vi "Place New Object After ID Object.vi"(7 "Named Cluster":variant, 8 "Identifying Attribute Value":string, 9 "Identifying Attribute Type":string, 10 "Element Type":string, 11 "XML String":string) -> (3 "Edited XML":string)   [LabVIEW 2019, in "EditSVG.lvclass"]
uses:
  EditSVG.lvclass
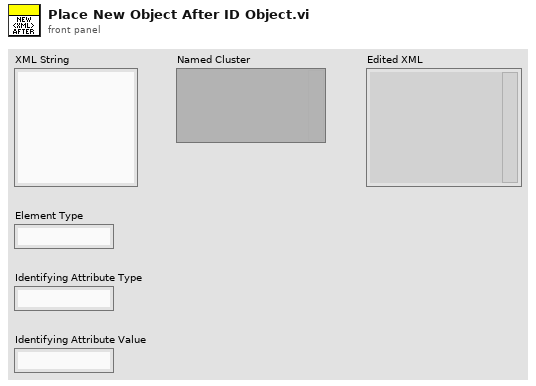
[diagram p1: front panel]
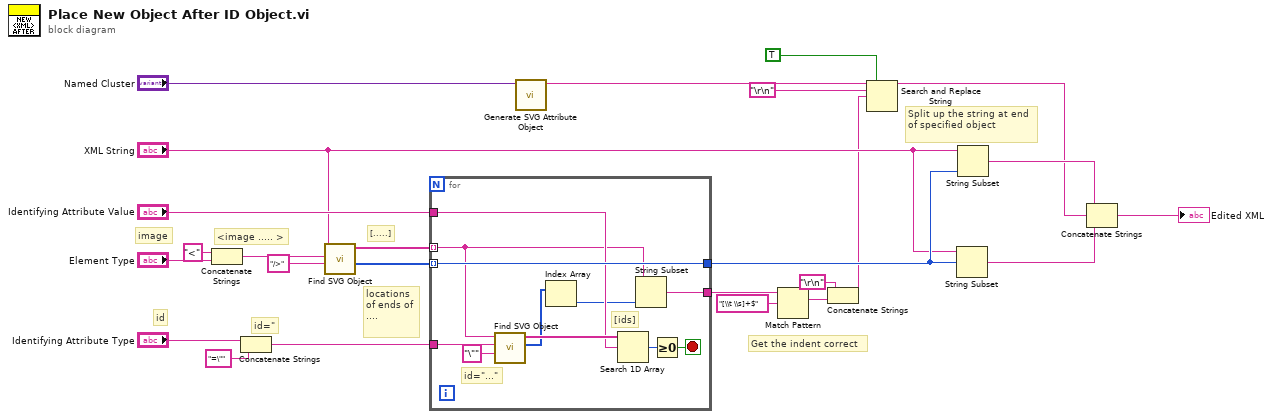
[diagram p0: block diagram]
diagram:
  # "Get the indent correct"
  # "Split up the string at end of specified object"
  # "id=\""
  # "id"
  # "locations of ends of ...."
  # "[.....]"
  # "<image ..... >"
  # "image"
  n1 = Concatenate Strings("<" ("string"), "Element Type") -> (w14:string)
  n2 = Concatenate Strings("Identifying Attribute Type", "=\"" ("string")) -> (w19:string)
  n3 = call "Find SVG Object.vi"("Ending Delimiter"="/>", "Beginning Delimiter"=w14, "XML String"="XML String") -> ("Ending Indices"=w17:i32[], "Found Values"=w24:string[])  [unwired: 6 in, 1 out]
  n4 = for {
    tunnel: w24 -> [w27] mode=indexing
    tunnel: w19 -> [w35]
    tunnel: "Identifying Attribute Value" -> [w30]
    tunnel: w17 -> [w34] mode=indexing
    tunnel: [w34] -> w13
    tunnel: [w26] -> w10
    stop <- w31 stop-if-true
    # "id=\"...\""
    # "[ids]"
    n5 = call "Find SVG Object.vi"("Ending Delimiter"="\"", "Beginning Delimiter"=w35, "XML String"=w27) -> ("Beginning Indices"=w29:i32[], "Found Values"=w33:string[])  [unwired: 6 in, 1 out]
    n6 = Index Array(array=w29) -> (element=w28:i32)  [unwired: 1 in]
    n7 = Search 1D Array(1D array=w33, element=w30) -> (index of element=w32:i32)  [unwired: 1 in]
    n8 = String Subset(string=w27, length (rest)=w28) -> (substring=w26:string)  [unwired: 1 in]
    n9 = Greater Or Equal To 0?(x=w32) -> (x >= 0?=w31:bool)
  }
  n10 = call "Generate SVG Attribute Object.vi"("Named Cluster of Data"="Named Cluster") -> ("SVG Attribute Object"=w3:string)  [unwired: 9 in, 1 out]
  n11 = Match Pattern(string=w10, regular expression="[\\t \\s]+$") -> (match substring=w7:string)  [unwired: 1 in, 3 out]
  n12 = Concatenate Strings("\r\n", w7) -> (w1:string)
  n13 = Search and Replace String(replace all?=TRUE ("replace all? (F)"), input string=w3, search string="\r\n", replace string=w1) -> (result string=w2:string)  [unwired: 4 in, 3 out]
  n14 = String Subset(string="XML String", offset (0)=w13) -> (substring=w23:string)  [unwired: 1 in]
  n15 = String Subset(string="XML String", length (rest)=w13) -> (substring=w12:string)  [unwired: 1 in]
  n16 = Concatenate Strings(w12, w2, w23) -> (→"Edited XML":string)
